vi "RT Functions v03a.vi"(7 "Function":T5(ring)=enum."Pulse On", 8 "error in (no error)":errorcluster, 9 "DAQ Trigger":T4={"Trig Source"=0, "Digital Trigger"=FALSE, "Trig Edge"=10171, "Pulse Line"=0, "Pulse On Time"=0} {"Pulse Line" items=["/Line0", "/Line1", "/Line2", "/Line3", "/Line4", "/Line5", "/Line6", "/Line7", "/Line8", "/Line9", "/Line10", "/Line11", "/Line12", "/Line13", "/Line14", "/Line15"]; "Trig Edge" items=["Rising"=10280, "Falling"=10171]; "Trig Source" items=["PFI0", "PFI1", "PFI2", "PFI3", "PFI4", "PFI5", "PFI6", "PFI7", "PFI8", "PFI9", "PFI10", "PFI11", "PFI12", "PFI13", "PFI14", "PFI15"]}, 10 "DAQ Timing":T3={"Number of Samples"=40000, "Samples Per Second"=970000.0, "Sample Mode"=10178, "Timeout (s)"=10.0} {"Sample Mode" items=["Continuous"=10123, "Finite Sample"=10178, "Hardware Timed Single Point"=12522]}, 11 "DAQ Channel":T2={"Channel"=1, "input terminal configuration"=10106, "Input Range Range"=10.0, "Device"="DAQ1"} {"input terminal configuration" items=["default"=-1, "RSE"=10083, "NRSE"=10078, "Differential"=10106, "Pseudodifferential"=12529]; "Input Range Range" items=["+/-10V"=10.0, "+/-5V"=5.0, "+/-2V"=2.0, "+/-1V"=1.0, "+/-0.5V"=0.5, "+/-0.2V"=0.2, "+/-0.1V"=0.1]; "Channel" items=["0"=0, "1"=1, "2"=2, "3"=3, "4"=4, "5"=5, "6"=6, "7"=7, "8"=8, "9"=9, "10"=10, "11"=11, "12"=12, "13"=13, "14"=14, "15"=15, "16"=16, "17"=18, "19"=20, "21"=22, "23"=24, "25"=26, "27"=28, "29"=30, "31"=32]}) -> (0 "error out":errorcluster, 2 "Wfm":waveform(dbl)={"t0"=timestamp(3404415606.9661703 s since 1904-01-01), "dt"=1.0299999999999546e-06, "Y"=array[1600 elements], "attributes"=variant("NI_ChannelName"=variant(string "Voltage"), "NI_UnitDescription"=variant(string "Volts"))}, 3 "Mean":dbl format="%0.2f", 6 "DAQ Pusle":T1)   [LabVIEW 2013]
uses:
  <vilib>/Analysis/baseanly.llb/Mean (DBL).vi
  <vilib>/Waveform/WDTOps.llb/WDT Get Waveform Subset DBL.vi
  <vilib>/Analysis/NI_AALBase.lvlib
panel:
  out "V3_Wfm":waveform(dbl)
  out "V2_Wfm":waveform(dbl)
  out "V1_Wfm":waveform(dbl)
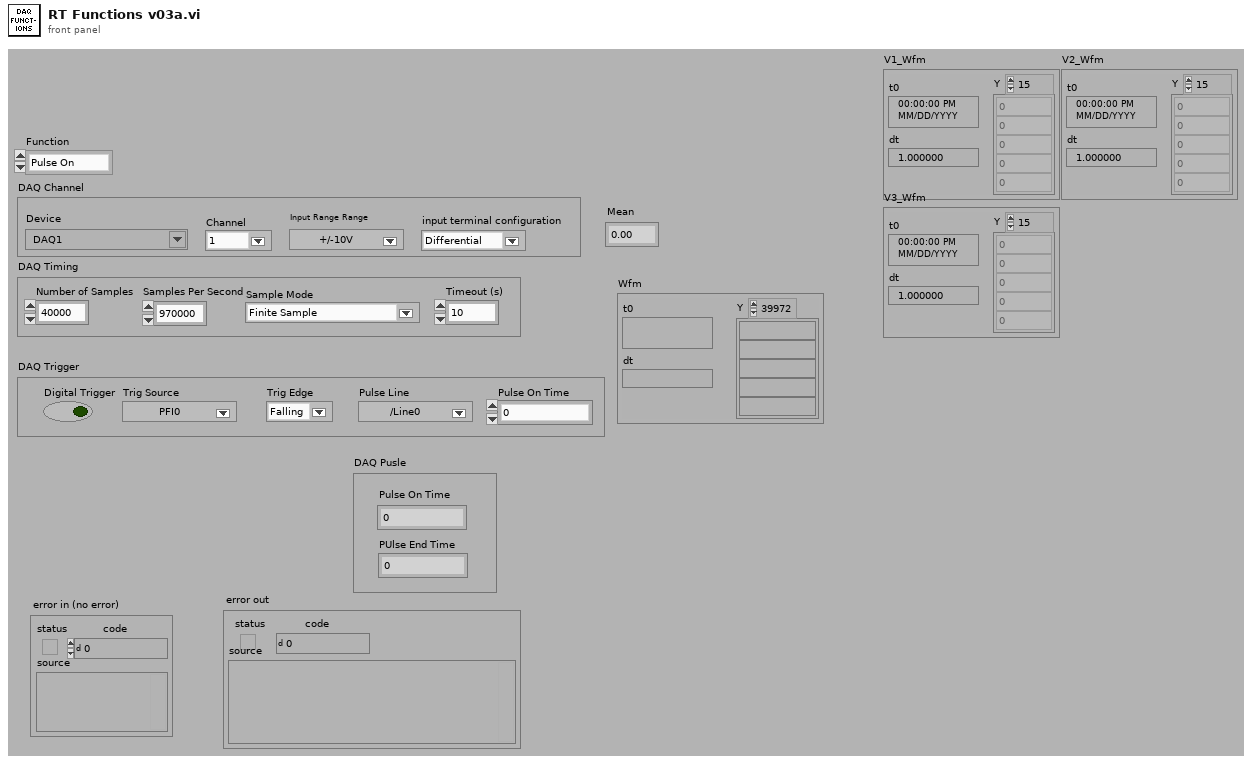
[diagram p1: front panel]
types:
  T1 = cluster{"Pulse On Time":u32, "PUlse End Time":u32}
  T2 = cluster{"Channel":u16, "input terminal configuration":i32, "Input Range Range":dbl, "Device":string}
  T3 = cluster{"Number of Samples":u32, "Samples Per Second":dbl, "Sample Mode":i32, "Timeout (s)":dbl}
  T4 = cluster{"Trig Source":u16, "Digital Trigger":bool, "Trig Edge":i32, "Pulse Line":u16, "Pulse On Time":u32}
  T5 = enum32{"V1 Measure", "V2 Measure", "V3 Measure", "Pulse On", "Pulse Off"}
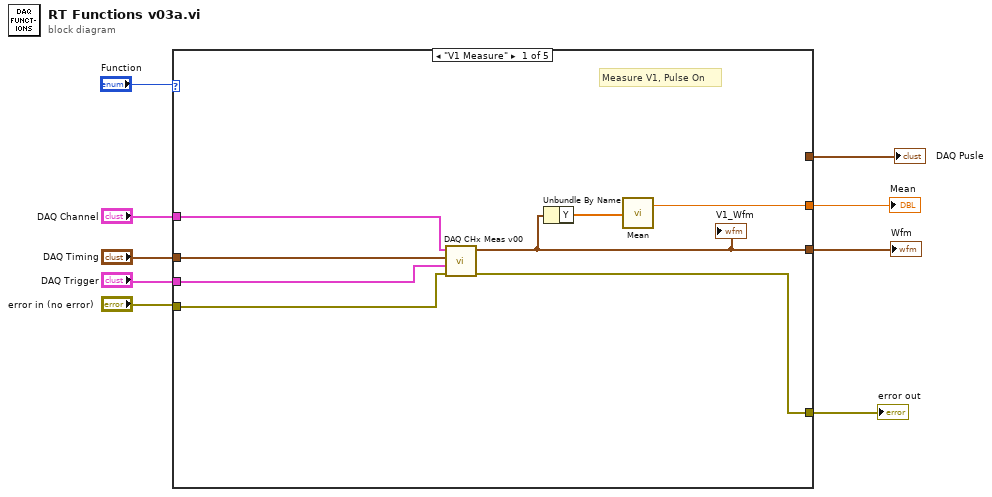
[diagram p0: block diagram]
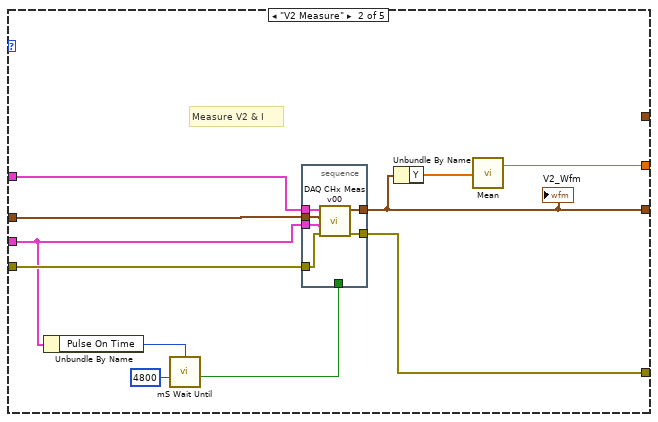
[diagram p2: hidden frame]
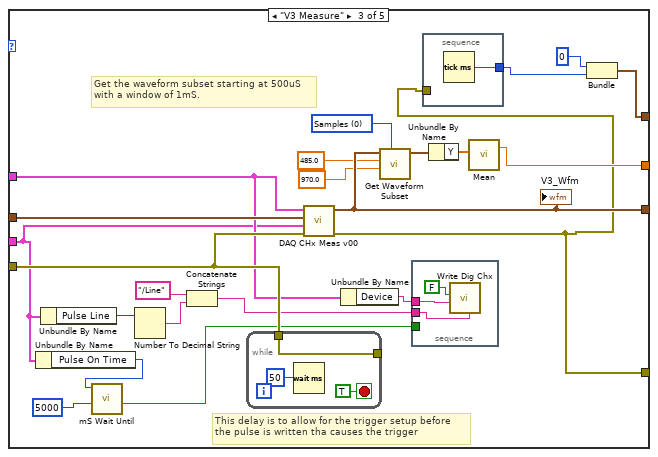
[diagram p3: hidden frame]
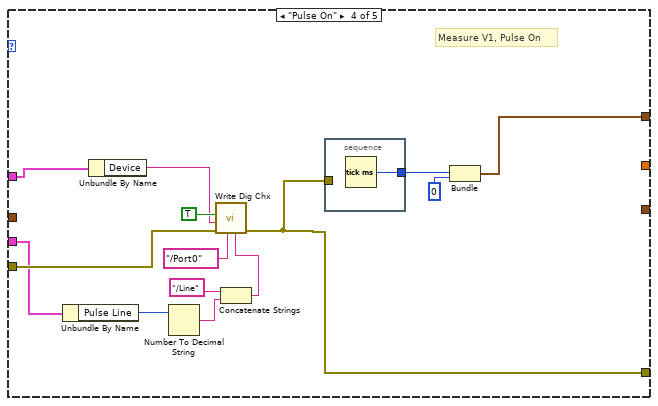
[diagram p4: hidden frame]
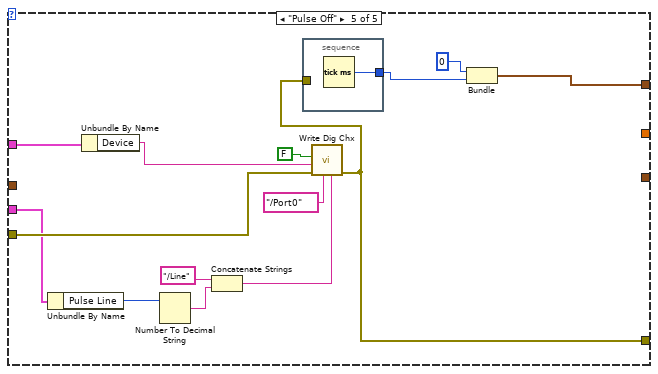
[diagram p5: hidden frame]
diagram:
  n1 = case shown="\"V1 Measure\"" "Function" {
    tunnel: "error in (no error)" -> [w17 w27 w54 w77 w92]
    tunnel: [w16 w28 w35 w73 w88] -> w8
    tunnel: "DAQ Channel" -> [w10 w22 w53 w76 w91]
    tunnel: "DAQ Timing" -> [w15 w26 w57 _ _]
    tunnel: "DAQ Trigger" -> [w14 w18 w39 w68 w83]
    tunnel: [w13 w24 w51 _ _] -> w3
    tunnel: [w11 w23 w55 _ _] -> w2
    tunnel: [_ _ w36 w65 w82] -> w1
    frame "V1 Measure" {
      # "Measure V1, Pulse On"
      n2 = call "DAQ CHx Meas v00.vi"("error in"=w17, "DAQ Trigger"=w14, "DAQ Timing"=w15, "DAQ Channel"=w10) -> ("error out"=w16:errorcluster, "Waveform"=w13:waveform(dbl))  [unwired: 6 in]
      "V1_Wfm" <- w13
      n3 = Unbundle By Name(w13) -> ("Y"=w12:dbl[])
      n4 = call-poly <vilib>:"Mean.vi"("X"=w12) -> ("mean"=w11:dbl)  [unwired: 1 out]
    }
    frame "V2 Measure" {
      # "Measure V2 & I"
      n5 = Unbundle By Name(w18) -> ("Pulse On Time"=w19:u32)
      n6 = call "mS Wait Until.vi"("mS Delta"=u16 4800, "mS Start Time"=w19) -> ("Done"=w20:bool)  [unwired: 8 in, 1 out]
      n7 = stacked-sequence {
        tunnel: [w34] -> w28
        tunnel: w27 -> [w33]
        tunnel: w26 -> [w32]
        tunnel: w18 -> [w31]
        tunnel: [w30] -> w24
        tunnel: w22 -> [w29]
        tunnel: w20 -> [_]
        frame #0 {
          n8 = call "DAQ CHx Meas v00.vi"("error in"=w33, "DAQ Trigger"=w31, "DAQ Timing"=w32, "DAQ Channel"=w29) -> ("error out"=w34:errorcluster, "Waveform"=w30:waveform(dbl))  [unwired: 6 in]
        }
      }
      "V2_Wfm" <- w24
      n9 = Unbundle By Name(w24) -> ("Y"=w25:dbl[])
      n10 = call-poly <vilib>:"Mean.vi"("X"=w25) -> ("mean"=w23:dbl)  [unwired: 1 out]
    }
    frame "V3 Measure" {
      w50 = u16 0 items=["Samples", "Relative Time"] ("start/duration format")
      # "Get the waveform subset starting at 500uS\nwith a window of 1mS."
      # "This delay is to allow for the trigger setup before\nthe pulse is written tha causes the trigger"
      n11 = Unbundle By Name(w39) -> ("Pulse On Time"=w44:u32)
      n12 = Unbundle By Name(w39) -> ("Pulse Line"=w43:u16)
      n13 = call "mS Wait Until.vi"("mS Delta"=u16 5000, "mS Start Time"=w44) -> ("Done"=w45:bool)  [unwired: 8 in, 1 out]
      n14 = Number To Decimal String(number=w43) -> (decimal integer string=w42:string)  [unwired: 1 in]
      n15 = Concatenate Strings("/Line", w42) -> (w40:string)
      n16 = while {
        tunnel: w54 -> [w62]
        tunnel: [w62] -> _
        stop <- TRUE stop-if-true
        n17 = Wait (ms)(milliseconds to wait=u32 50) -> ()  [unwired: 1 out]
      }
      n18 = call "DAQ CHx Meas v00.vi"("error in"=w54, "DAQ Trigger"=w39, "DAQ Timing"=w57, "DAQ Channel"=w53) -> ("error out"=w35:errorcluster, "Waveform"=w51:waveform(dbl))  [unwired: 6 in]
      "V3_Wfm" <- w51
      n19 = Unbundle By Name(w53) -> ("Device"=w52:string)
      n20 = call-poly <vilib>:"Get Waveform Subset.vi"("start/duration format"=w50, "duration"=970.0, "start samples/time"=485.0, "waveform in"=w51) -> ("waveform out"=w47:waveform(dbl))  [unwired: 2 in, 3 out]
      n21 = stacked-sequence {
        tunnel: w52 -> [w60]
        tunnel: w40 -> [w59]
        tunnel: w45 -> [_]
        frame #0 {
          n22 = call "Write Dig Chx.vi"("Line"=w59, "Device"=w60, "Ch Value"=FALSE) -> ()  [unwired: 8 in, 1 out]
        }
      }
      n23 = stacked-sequence {
        tunnel: [w58] -> w37
        tunnel: w35 -> [_]
        frame #0 {
          n24 = Tick Count (ms)() -> (millisecond timer value=w58:u32)
        }
      }
      n25 = Unbundle By Name(w47) -> ("Y"=w56:dbl[])
      n26 = call-poly <vilib>:"Mean.vi"("X"=w56) -> ("mean"=w55:dbl)  [unwired: 1 out]
      n27 = Bundle(u32 0, "millisecond timer value"=w37) -> (w36:cluster{u32, "millisecond timer value":u32})  [unwired: 1 in]
    }
    frame "Pulse On" {
      # "Measure V1, Pulse On"
      n28 = Unbundle By Name(w68) -> ("Pulse Line"=w70:u16)
      n29 = Unbundle By Name(w76) -> ("Device"=w75:string)
      n30 = Number To Decimal String(number=w70) -> (decimal integer string=w71:string)  [unwired: 1 in]
      n31 = Concatenate Strings("/Line", w71) -> (w69:string)
      n32 = call "Write Dig Chx.vi"("Line"=w69, "Port"="/Port0", "error in"=w77, "Device"=w75, "Ch Value"=TRUE) -> ("error out"=w73:errorcluster)  [unwired: 6 in]
      n33 = stacked-sequence {
        tunnel: w73 -> [_]
        tunnel: [w79] -> w67
        frame #0 {
          n34 = Tick Count (ms)() -> (millisecond timer value=w79:u32)
        }
      }
      n35 = Bundle("millisecond timer value"=w67, u32 0) -> (w65:cluster{"millisecond timer value":u32, u32})  [unwired: 1 in]
    }
    frame "Pulse Off" {
      n36 = Unbundle By Name(w83) -> ("Pulse Line"=w85:u16)
      n37 = Unbundle By Name(w91) -> ("Device"=w90:string)
      n38 = Number To Decimal String(number=w85) -> (decimal integer string=w86:string)  [unwired: 1 in]
      n39 = Concatenate Strings("/Line", w86) -> (w84:string)
      n40 = call "Write Dig Chx.vi"("Line"=w84, "Port"="/Port0", "error in"=w92, "Device"=w90, "Ch Value"=FALSE) -> ("error out"=w88:errorcluster)  [unwired: 6 in]
      n41 = stacked-sequence {
        tunnel: w88 -> [_]
        tunnel: [w94] -> w81
        frame #0 {
          n42 = Tick Count (ms)() -> (millisecond timer value=w94:u32)
        }
      }
      n43 = Bundle(u32 0, "millisecond timer value"=w81) -> (w82:cluster{u32, "millisecond timer value":u32})  [unwired: 1 in]
    }
  }
  "error out" <- w8
  "Wfm" <- w3
  "Mean" <- w2
  "DAQ Pusle" <- w1
